vi "Create Measurement Client.vi"() -> ()   [LabVIEW 2021, in "MeasurementClient Editor.lvlib"]
uses:
  _MeasurementClient Utility/MeasurementClient Editor.lvlib
  <vilib>/Utility/error.llb/ErrWarn.ctl
  _MeasurementClient Utility/Refresh Button.ctl
  <vilib>/gRPC/Generated APIs/ni/measurementlink/discovery/v1/RPC Messages/ni_measurementlink_discovery_v1_EnumerateServicesRequest.ctl
  _MeasurementClient Utility/Data Holder.ctl
  <vilib>/gRPC/Generated APIs/ni/measurementlink/discovery/v1/RPC Messages/ni_measurementlink_discovery_v1_EnumerateServicesResponse.ctl
  <vilib>/gRPC/Generated APIs/ni/measurementlink/discovery/v1/RPC Messages/ni_measurementlink_discovery_v1_ServiceDescriptor.ctl
  <vilib>/gRPC/Generated APIs/ni/measurementlink/discovery/v1/RPC Messages/ni_measurementlink_discovery_v1_ServiceDescriptor_AnnotationsEntry.ctl
  <vilib>/Utility/miscctls.llb/LVRowAndColumnTypeDef.ctl
  _Generator Helpers/Generator Helpers.lvlib
  <vilib>/gRPC/Generated APIs/ni/measurementlink/discovery/v1/ni.measurementlink.discovery.v1.api.lvlib
  <vilib>/Plug-In SDKs/Clients/Discovery V1/NI Discovery V1 Client.lvlib
  Measurement V2 Client Generator Runtime/NI Measurement V2 Client Generator Runtime.lvlib
panel:
  in  "Tab Control":enum32{"Inputs", "Status"}(tab)
  in  "Select All":bool
  in  "Refresh":T1
  out "Active Project Name":string
  in  "Available Measurements":i32(listbox)=-1
  in  "Create Client":bool
  out "Warning":T2 caption="The selected measurement plug-in client name(s) already exists or contains invalid characters: \n \\ / : * ? \" < > |"
  out "Error Message":string
  in  "Client Status":i32(listbox)=-1 caption="Measurement Plug-In Client Creation Status"
  # "* Project in which the measurement plug-in client vi will be created"
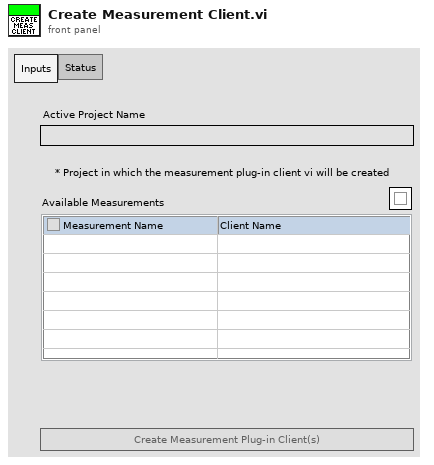
[diagram p1: front panel]
types:
  T1 = typedef "MeasurementClient Editor.lvlib/Refresh Button.ctl" = bool
  T2 = typedef "ErrWarn.ctl" = bool
  T3 = enum8{"Enabled", "Disabled", "Disabled and Grayed Out"}
  T4 = typedef "MeasurementClient Editor.lvlib/Data Holder.ctl" = cluster{"project ref":refnum<vi>, "multicolumnListbox ref":refnum<vi>, "available measurement details":T5, "statusListbox ref":refnum<vi>, "error messages":string[]}
  T5 = typedef "ni.measurementlink.discovery.v1.api.lvlib/ni_measurementlink_discovery_v1_EnumerateServicesResponse.ctl" = cluster{"available_services":T6[], "unreachable":string[]}
  T6 = typedef "ni.measurementlink.discovery.v1.api.lvlib/ni_measurementlink_discovery_v1_ServiceDescriptor.ctl" = cluster{"display_name":string, "description_url":string, "provided_interfaces":string[], "service_class":string, "annotations":T7[], "versions":string[]}
  T7 = typedef "ni.measurementlink.discovery.v1.api.lvlib/ni_measurementlink_discovery_v1_ServiceDescriptor_AnnotationsEntry.ctl" = cluster{"key":string, "value":string}
  T8 = typedef "ni.measurementlink.discovery.v1.api.lvlib/ni_measurementlink_discovery_v1_EnumerateServicesRequest.ctl" = cluster{"provided_interface":string, "service_class":string}
  T9 = typedef "LVRowAndColumnTypeDef.ctl" = cluster{"Row":i32, "Column":i32}
  T10 = typedef "MeasurementClient Editor.lvlib/Client Creation Status.ctl" = enum16{"Success", "Fail"}
  T11 = typedef "LVPoint32TypeDef.ctl" = cluster{"Horizontal":i32, "Vertical":i32}
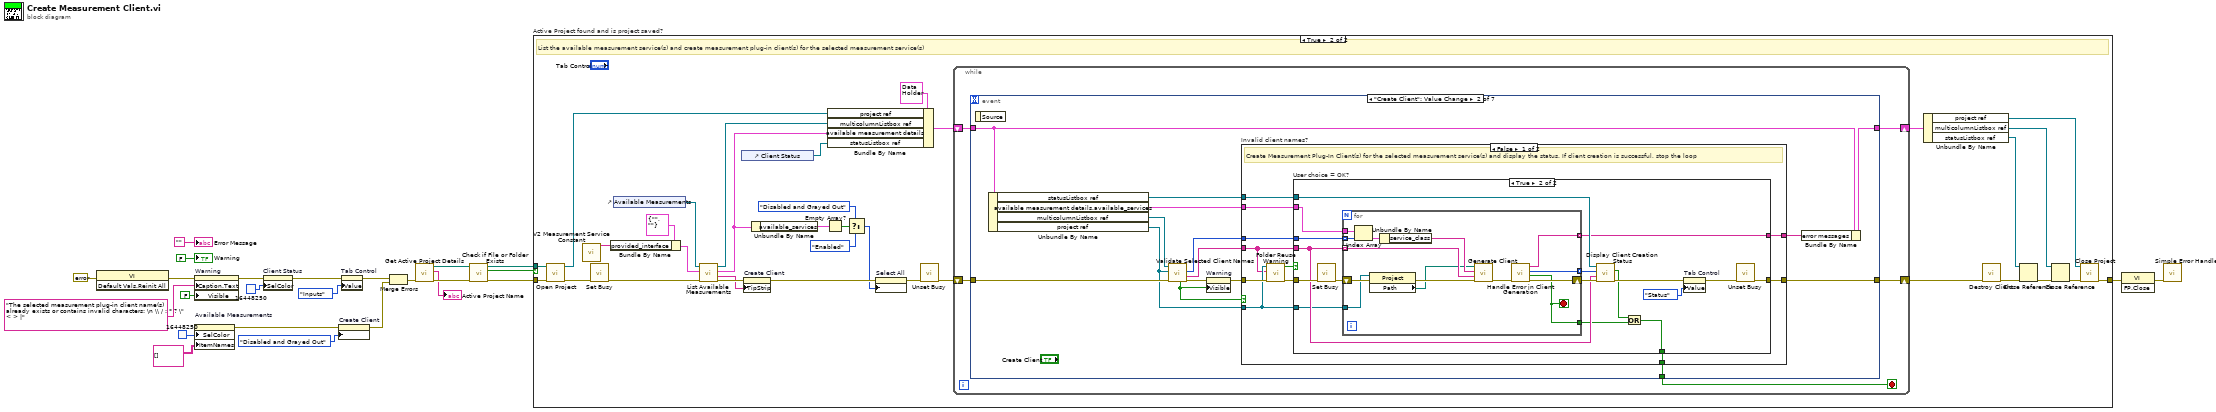
[diagram p0: block diagram]
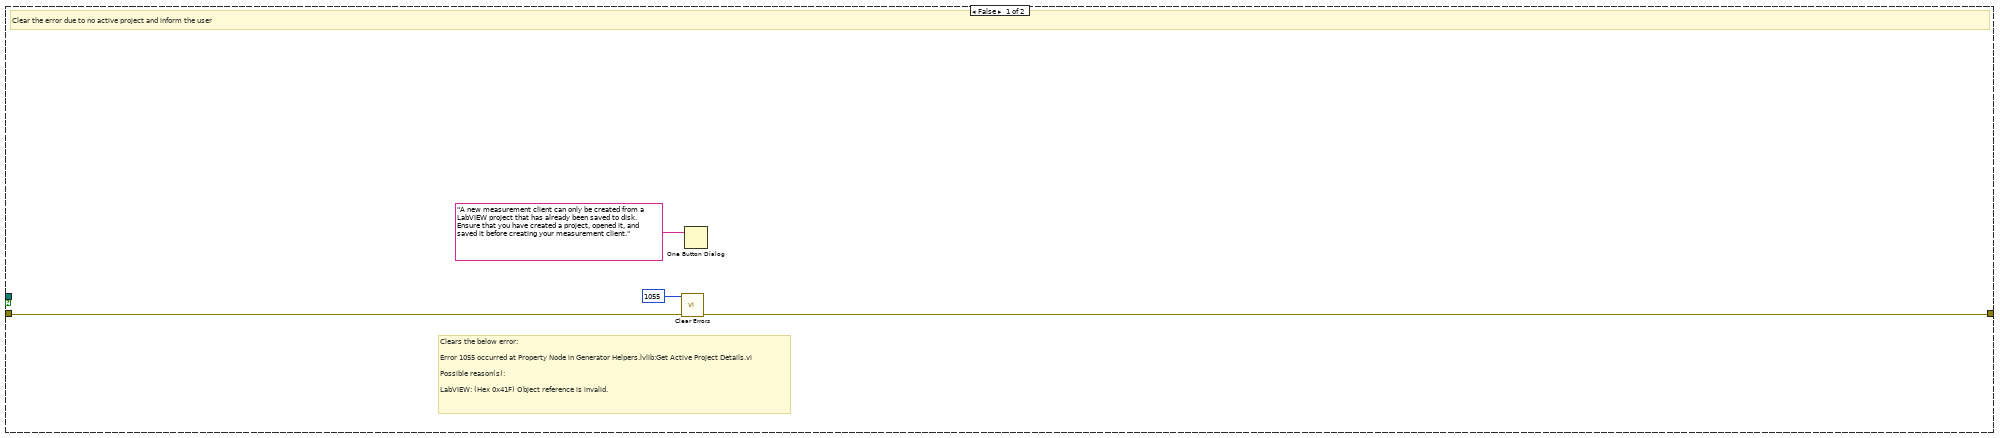
[diagram p2: hidden frame]
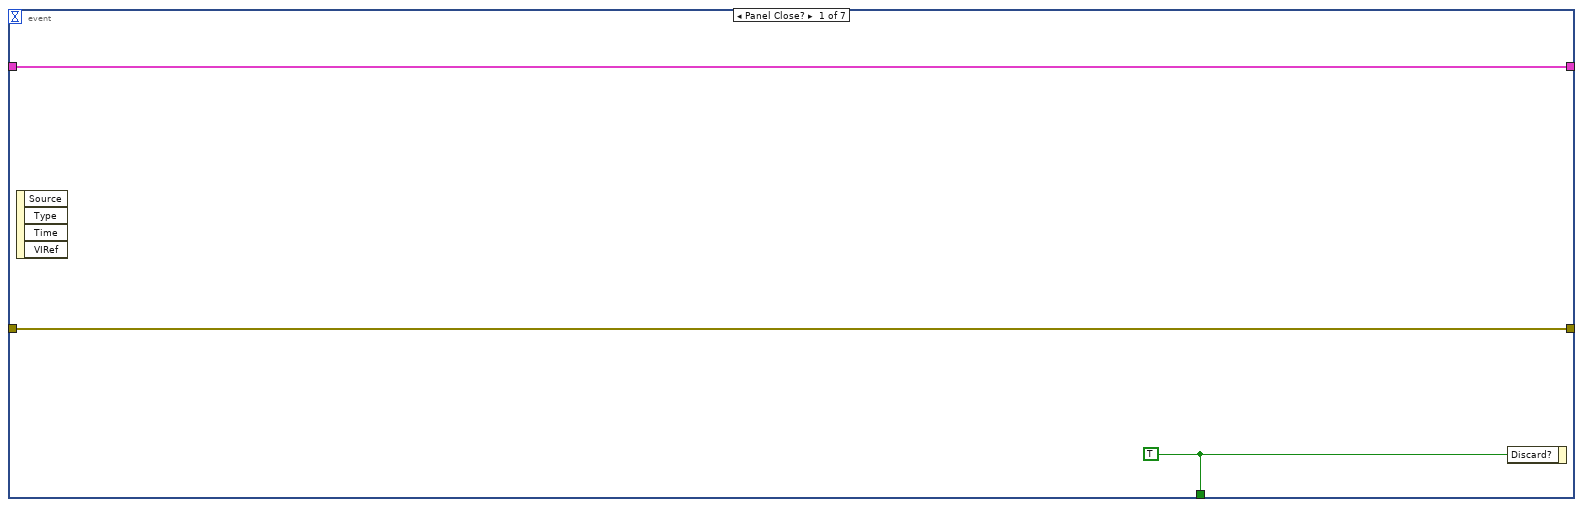
[diagram p3: hidden frame]
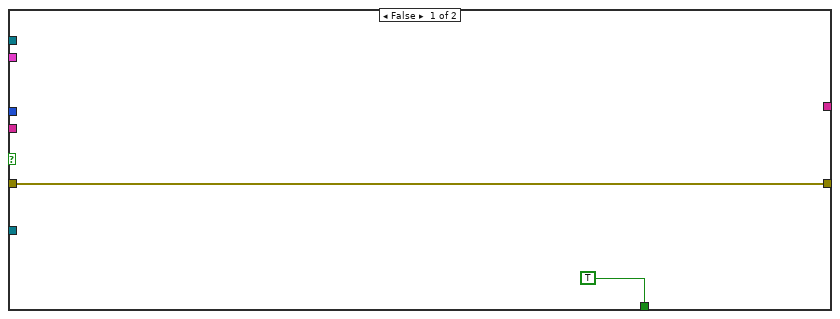
[diagram p4: hidden frame]
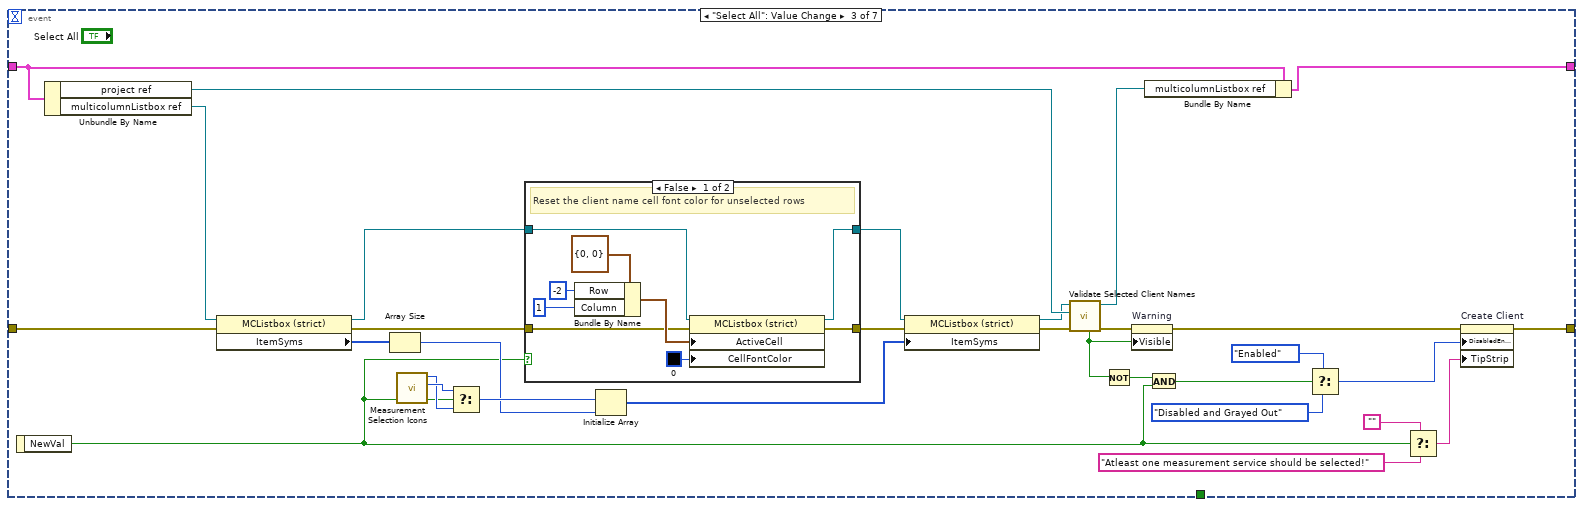
[diagram p6: hidden frame]
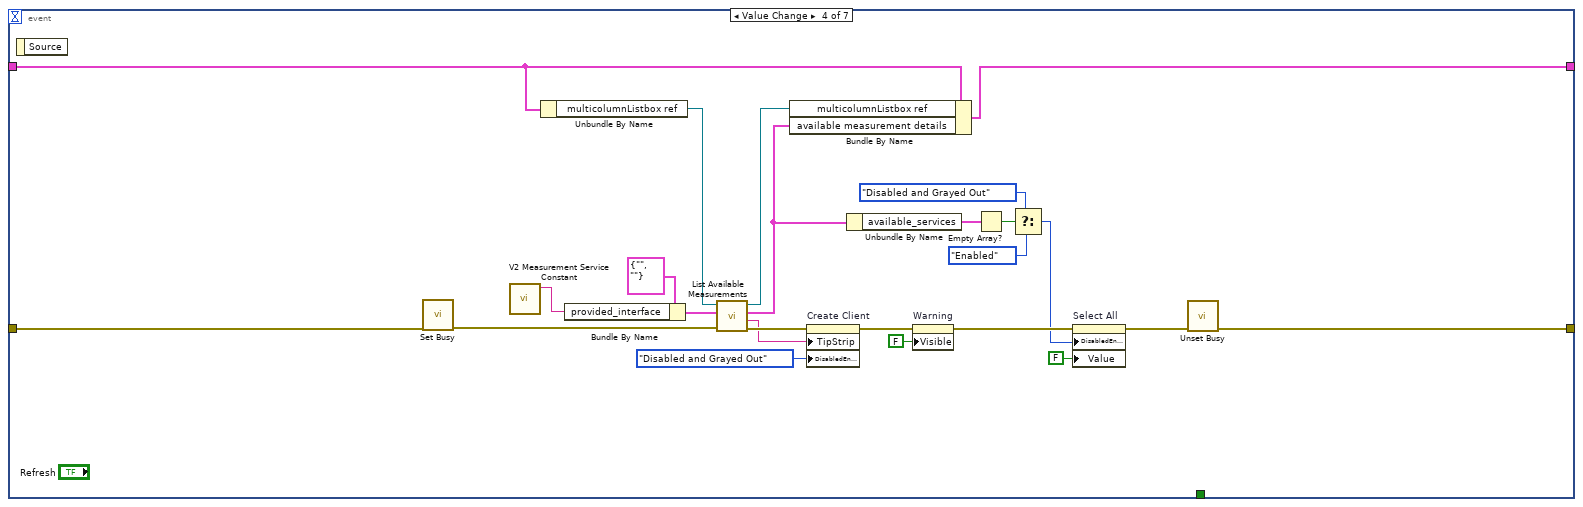
[diagram p8: hidden frame]
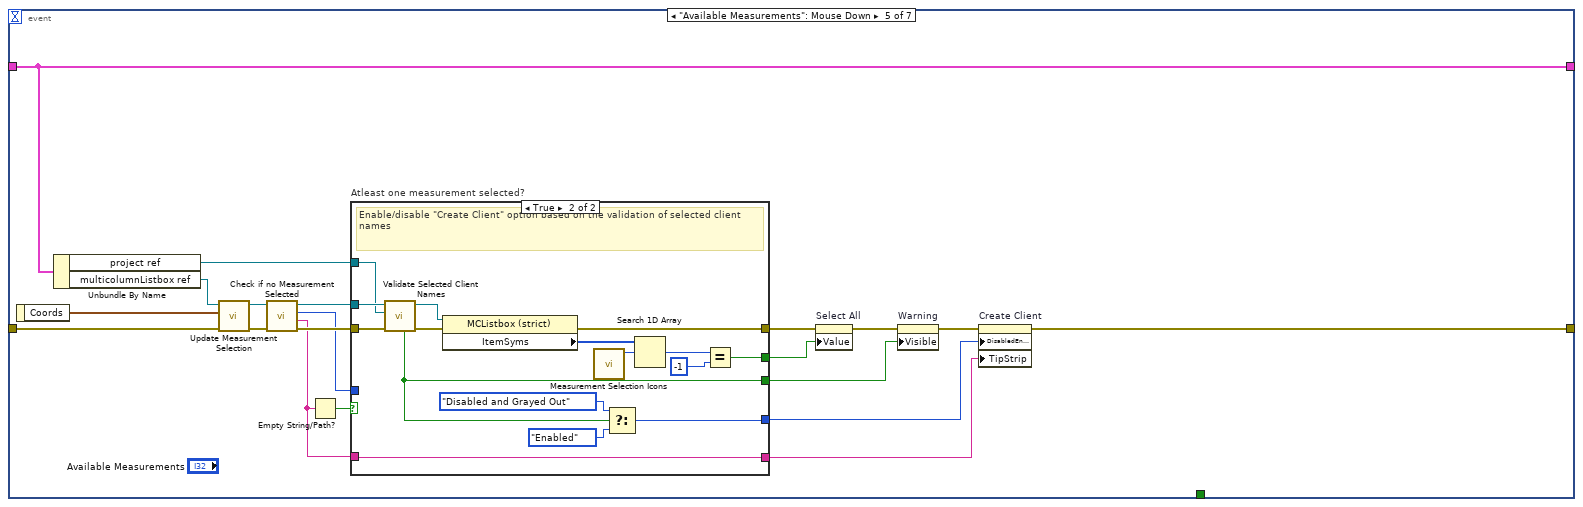
[diagram p9: hidden frame]
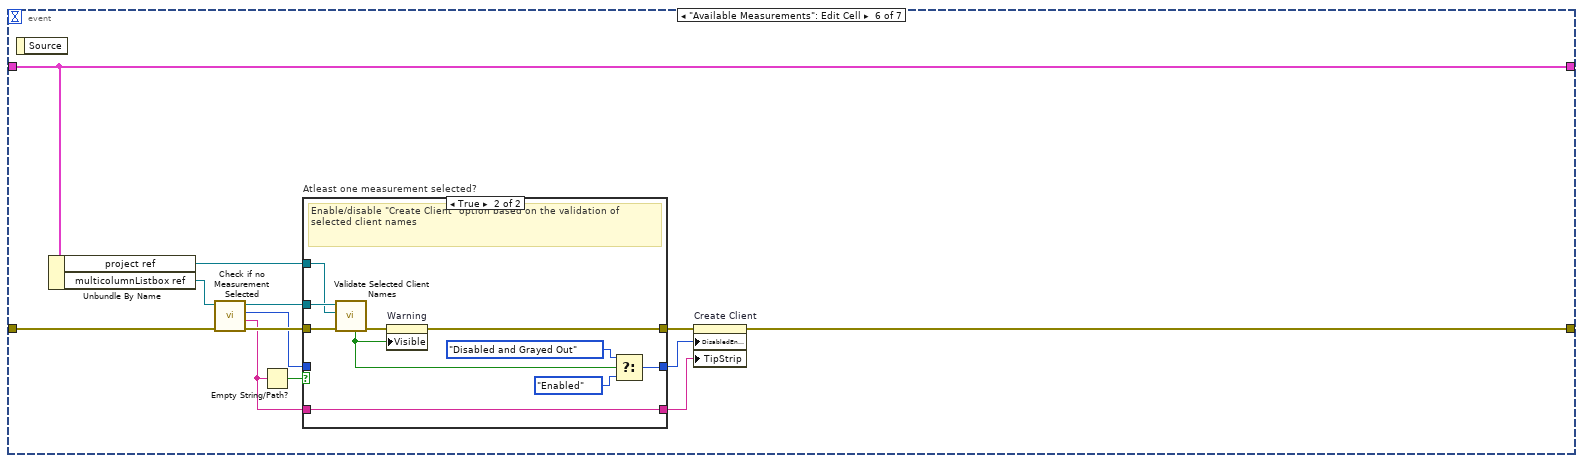
[diagram p11: hidden frame]
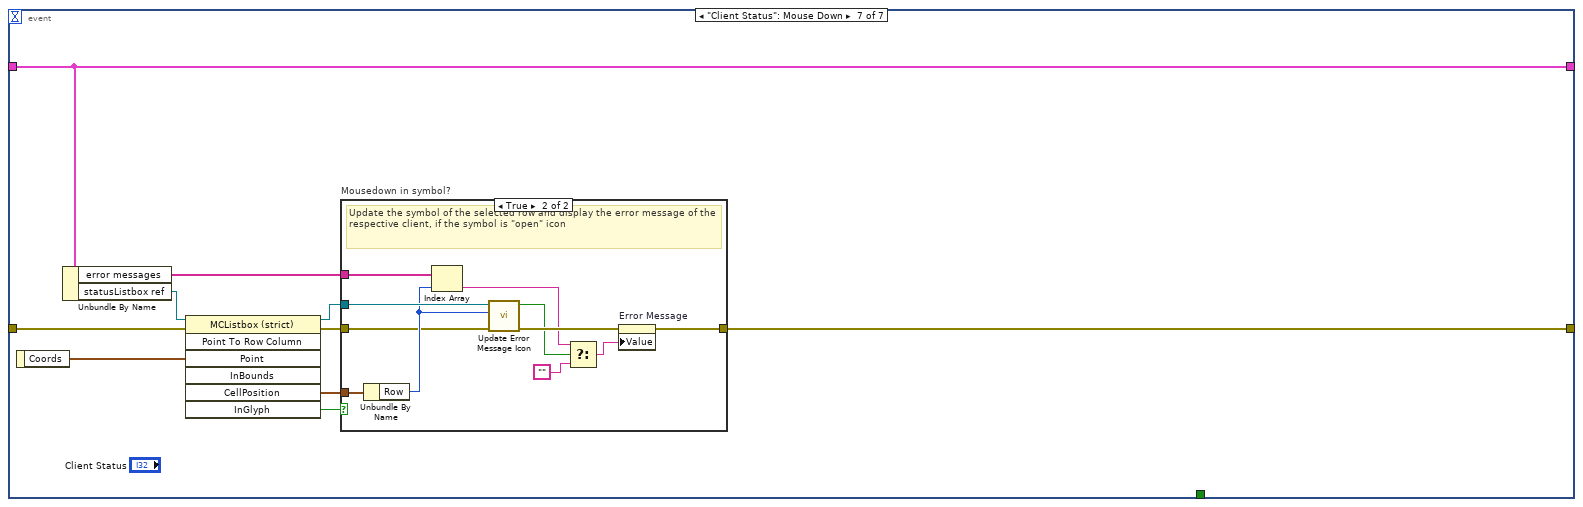
[diagram p13: hidden frame]
diagram:
  n1 = invoke class="VI" method="Default Vals.Reinit All"(error in=errorcluster {"status"=FALSE, "code"=0, "source"=""} ("error in (no error)")) -> (error out=w19:errorcluster)  [unwired: 2 in, 2 out]
  n2 = property on="Warning" class="Bool"(error in=w19, "Caption.Text"="The selected measurement plug-in client name(s) already exists or contains invalid characters: \n \\ / : * ? \" < > |" ("Status"), "Visible"=FALSE) -> (error out=w12:errorcluster)  [unwired: 1 in, 1 out]
  n3 = property on="Available Measurements" class="MCListbox (strict)"("SelColor"=u32 16448250 ("Selection Color"), "ItemNames"=string[][] [] ("Item Names")) -> (error out=w9:errorcluster)  [unwired: 2 in, 1 out]
  n4 = property on="Client Status" class="MCListbox (strict)"(error in=w12, "SelColor"=u32 16448250 ("Selection Color")) -> (error out=w13:errorcluster)  [unwired: 1 in, 1 out]
  n5 = property on="Create Client" class="Bool"(error in=w9, "DisabledEnum"=T3."Disabled and Grayed Out" ("Disabled")) -> (error out=w8:errorcluster)  [unwired: 1 in, 1 out]
  n6 = property on="Tab Control" class="TabCtl (strict)"(error in=w13, "Value"=enum32{"Inputs", "Status"}."Inputs" ("Tab Control")) -> (error out=w11:errorcluster)  [unwired: 1 in, 1 out]
  n7 = Merge Errors(w11, w8) -> (w7:errorcluster)
  n8 = call "Get Active Project Details.vi"("error in"=w7) -> ("error out"=w6:errorcluster, "name"=→"Active Project Name":string, "path"=w5:path)  [unwired: 8 in]
  n9 = call <vilib>:"Check if File or Folder Exists.vi"("error in (no error)"=w6, "path"=w5) -> ("error out"=w2:errorcluster, "file or folder exists?"=w1:bool, "dup path"=w3:path)  [unwired: 7 in]
  n10 = case "Active Project found and is project saved?" shown="True" w1 {
    tunnel: [w29 w47] -> w23
    tunnel: w3 -> [_ w62]
    tunnel: w2 -> [w26 w56]
    frame False {
      # "Clears the below error:\n\nError 1055 occurred at Property Node in Generator Helpers.lvlib:Get Active Project Details.vi\n\nPossible reason(s):\n\nLabVIEW: (Hex 0x41F) Object reference is invalid."
      # "Clear the error due to no active project and inform the user"
      n11 = call <vilib>:"Clear Errors.vi"("error in (no error)"=w26, "specific error code to clear (0: all)"=1055) -> ("error out"=w29:errorcluster)  [unwired: 4 in, 1 out]
      n12 = One Button Dialog(message="A new measurement client can only be created from a LabVIEW project that has already been saved to disk.  Ensure that you have created a project, opened it, and saved it before creating your measurement client.") -> ()  [unwired: 1 in, 1 out]
    }
    frame True {
      # "List the available measurement service(s) and create measurement plug-in client(s) for the selected measurement service(s)"
      n13 = call "Open Project.vi"("error in"=w56, "path"=w62) -> ("error out"=w57:errorcluster, "project ref"=w51:refnum<vi>)  [unwired: 8 in]
      n14 = call "V2 Measurement Service Constant.vi"() -> ("provided_interface"=w39:string)  [unwired: 11 in]
      n15 = call <vilib>:"Set Busy.vi"("error in (no error)"=w57) -> ("error out"=w59:errorcluster)  [unwired: 9 in, 1 out]
      n16 = Bundle By Name(cluster=T8 {"provided_interface"="", "service_class"=""} ("request data"), "provided_interface"=w39) -> (w40:T8)
      n17 = control-ref of="Available Measurements"() -> (w49:refnum<vi>)
      n18 = call "List Available Measurements.vi"("error in (no error)"=w59, "enumerate services request"=w40, "multicolumnListbox ref in"=w49) -> ("error out"=w60:errorcluster, "warning"=w53:string, "available measurement details"=w36:T5, "multicolumnListbox ref"=w50:refnum<vi>)  [unwired: 5 in]
      n19 = control-ref of="Client Status"() -> (w30:refnum<vi>)
      n20 = property on="Create Client" class="Bool"(error in=w60, "TipStrip"=w53) -> (error out=w38:errorcluster)  [unwired: 1 in, 1 out]
      n21 = Unbundle By Name(w36) -> ("available_services"=w35:T6[])
      n22 = Empty Array?(array=w35) -> (empty?=w32:bool)
      n23 = Bundle By Name(cluster=T4 {"project ref"=refnum, "multicolumnListbox ref"=refnum, "available measurement details"={"available_services"=[], "unreachable"=[]}, "statusListbox ref"=refnum, "error messages"=[]}, "project ref"=w51, "multicolumnListbox ref"=w50, "available measurement details"=w36, "statusListbox ref"=w30) -> (w48:T4)
      n24 = Select(t=T3."Disabled and Grayed Out" ("Disabled"), s=w32, f=T3."Enabled" ("Disabled")) -> (s? t:f=w31:T3)
      n25 = property on="Select All" class="Bool (strict)"(error in=w38, "DisabledEnum"=w31) -> (error out=w37:errorcluster)  [unwired: 1 in, 1 out]
      n26 = call <vilib>:"Unset Busy.vi"("error in (no error)"=w37) -> ("error out"=w58:errorcluster)  [unwired: 10 in]
      n27 = while {
        shift-right: [w66] -> w43
        shift-left: w58 -> [w67]
        shift-right: [w64] -> w54
        shift-left: w48 -> [w65]
        stop <- w63 stop-if-true
        n28 = event shown="[1] \"Create Client\": Value Change" {
          selector: _ -> [_ _ _ _ _ _ _]
          dyn-events: _ -> [_ _ _ _ _ _ _]
          timeout: _ -> [_ _ _ _ _ _ _]
          tunnel: w67 -> [w70 w85 w140 w185 w211 w237 w268]
          tunnel: [w70 w75 w149 w182 w210 w247 w271] -> w66
          tunnel: w65 -> [w69 w80 w147 w193 w216 w248 w269]
          tunnel: [w69 w77 w145 w191 w216 w248 w269] -> w64
          tunnel: [w68 w72 _ _ _ _ _] -> w63
          event Panel Close? {
            w68 = TRUE ("Discard?")
            # "Discard panel close and stop the execution of measurement plug-in client generator"
            n29 = event-data() -> ()  [unwired: 1 in, 4 out]
            n30 = event-data("Discard?"=w68) -> ()  [unwired: 1 in, 1 out]
          }
          event "Create Client": Value Change {
            # "Validate client name and create measurement plug-in client for the selected measurement service(s), if no invalid client name"
            n31 = event-data() -> ()  [unwired: 1 in, 1 out]
            n32 = Unbundle By Name(w80) -> ("statusListbox ref"=w78:refnum<vi>, "available measurement details.available_services"=w76:T6[], "multicolumnListbox ref"=w84:refnum<vi>, "project ref"=w79:refnum<vi>)
            n33 = call "Validate Selected Client Names.vi"("error in (no error)"=w85, "project ref"=w79, "multicolumnListbox in"=w84) -> ("error out"=w83:errorcluster, "selected client names"=w74:string[], "selected measurement indices"=w81:i32[], "warning?"=w73:bool)  [unwired: 4 in, 1 out]
            n34 = property on="Warning" class="Bool"(error in=w83, "Visible"=w73) -> (error out=w82:errorcluster)  [unwired: 1 in, 1 out]
            n35 = case "Invalid client names?" shown="False" w73 {
              tunnel: w82 -> [w96 w130]
              tunnel: w81 -> [w95 _]
              tunnel: w79 -> [w89 _]
              tunnel: [w92 w130] -> w75
              tunnel: w78 -> [w94 _]
              tunnel: w76 -> [w93 _]
              tunnel: w74 -> [w87 _]
              tunnel: [w91 _] -> w72
              tunnel: [w86 _] -> w71
              frame False {
                # "Create Measurement Plug-In Client(s) for the selected measurement service(s) and display the status. If client creation is successful, stop the loop"
                n36 = call "Folder Reuse Warning.vi"("error in"=w96, "folder names"=w87, "project ref"=w89) -> ("error out"=w90:errorcluster, "proceed?"=w88:bool)  [unwired: 7 in]
                n37 = case "User choice = OK?" shown="True" w88 {
                  tunnel: w95 -> [_ w115]
                  tunnel: w94 -> [_ w112]
                  tunnel: w93 -> [_ w111]
                  tunnel: [w98 w107] -> w92
                  tunnel: [TRUE ("all success?") w102] -> w91
                  tunnel: w90 -> [w98 w106]
                  tunnel: w87 -> [_ w105]
                  tunnel: w89 -> [_ w104]
                  tunnel: [_ w99] -> w86
                  frame False {
                  }
                  frame True {
                    n38 = call <vilib>:"Set Busy.vi"("error in (no error)"=w106) -> ("error out"=w114:errorcluster)  [unwired: 9 in, 1 out]
                    n39 = for {
                      tunnel: w111 -> [w129]
                      shift-right: [w119] -> w113
                      shift-left: w114 -> [w126]
                      tunnel: w115 -> [w127] mode=indexing
                      tunnel: w104 -> [w122]
                      tunnel: w105 -> [w124] mode=indexing
                      tunnel: [w118] -> w99 mode=indexing
                      tunnel: [w117] -> w101 mode=indexing
                      tunnel: [w116] -> w100
                      stop <- w116 stop-if-true
                      n40 = Index Array(array=w129, index=w127) -> (element=w128:T6)
                      n41 = property class="Project"(reference=w122, error in=w126) -> (error out=w123:errorcluster, "Path"=w121:path)  [unwired: 1 out]
                      n42 = Unbundle By Name(w128) -> ("service_class"=w125:string)
                      n43 = call "Generate Client.vi"("error in"=w123, "client name"=w124, "service class"=w125, "project path"=w121) -> ("error out"=w120:errorcluster)  [unwired: 7 in]
                      n44 = call "Handle Error in Client Generation.vi"("error in"=w120) -> ("error out"=w119:errorcluster, "InstrumentStudio Pro < Q4?"=w116:bool, "status"=w117:T10, "error message"=w118:string)  [unwired: 7 in]
                    }
                    n45 = call "Display Client Creation Status.vi"("error in"=w113, "client names"=w105, "status"=w101, "statusListbox in"=w112) -> ("error out"=w109:errorcluster, "all success?"=w103:bool)  [unwired: 5 in, 1 out]
                    n46 = Or(x=w103, y=w100) -> (x .or. y?=w102:bool)
                    n47 = property on="Tab Control" class="TabCtl (strict)"(error in=w109, "Value"=enum32{"Inputs", "Status"}."Status" ("Tab Control")) -> (error out=w108:errorcluster)  [unwired: 1 in, 1 out]
                    n48 = call <vilib>:"Unset Busy.vi"("error in (no error)"=w108) -> ("error out"=w107:errorcluster)  [unwired: 10 in]
                  }
                }
              }
              frame True {
                # "Pass"
              }
            }
            n49 = Bundle By Name(cluster=w80, "error messages"=w71) -> (w77:T4)
          }
          event "Select All": Value Change {
            n50 = event-data() -> ("NewVal"=w132:bool)  [unwired: 1 in]
            n51 = Unbundle By Name(w147) -> ("project ref"=w148:refnum<vi>, "multicolumnListbox ref"=w161:refnum<vi>)
            n52 = property class="MCListbox (strict)"(reference=w161, error in=w140) -> (reference out=w144:refnum<vi>, error out=w139:errorcluster, "ItemSyms"=w135:i32[])
            n53 = Array Size(array=w135) -> (size(s)=w133:i32)
            n54 = call "Measurement Selection Icons.vi"() -> ("Checked"=w137:i32, "Unchecked"=w136:i32)  [unwired: 10 in]
            n55 = Select(t=w137, s=w132, f=w136) -> (s? t:f=w134:i32)
            n56 = case shown="False" w132 {
              tunnel: w144 -> [w166 w172]
              tunnel: [w165 w172] -> w142
              tunnel: w139 -> [w164 w171]
              tunnel: [w163 w171] -> w138
              frame False {
                # "Reset the client name cell font color for unselected rows"
                n57 = Bundle By Name(cluster=T9 {"Row"=0, "Column"=0} ("Active Cell:Active Cell"), "Row"=-2, "Column"=1) -> (w168:T9)
                n58 = property class="MCListbox (strict)"(reference=w166, error in=w164, "ActiveCell"=w168, "CellFontColor"=u32 0 ("Active Cell:Cell Font:Color")) -> (reference out=w165:refnum<vi>, error out=w163:errorcluster)
              }
              frame True {
                # "Pass"
              }
            }
            n59 = Initialize Array(w134, w133) -> (w131:i32[])
            n60 = property class="MCListbox (strict)"(reference=w142, error in=w138, "ItemSyms"=w131) -> (reference out=w141:refnum<vi>, error out=w143:errorcluster)
            n61 = call "Validate Selected Client Names.vi"("error in (no error)"=w143, "project ref"=w148, "multicolumnListbox in"=w141) -> ("error out"=w160:errorcluster, "multicolumnListbox out"=w146:refnum<vi>, "warning?"=w158:bool)  [unwired: 4 in, 2 out]
            n62 = Not(x=w158) -> (.not. x?=w157:bool)
            n63 = property on="Warning" class="Bool"(error in=w160, "Visible"=w158) -> (error out=w159:errorcluster)  [unwired: 1 in, 1 out]
            n64 = Bundle By Name(cluster=w147, "multicolumnListbox ref"=w146) -> (w145:T4)
            n65 = And(x=w157, y=w132) -> (x .and. y?=w156:bool)
            n66 = Select(t=T3."Enabled" ("Disabled"), s=w156, f=T3."Disabled and Grayed Out" ("Disabled")) -> (s? t:f=w153:T3)
            n67 = Select(t="", s=w132, f="Atleast one measurement service should be selected!") -> (s? t:f=w150:string)
            n68 = property on="Create Client" class="Bool"(error in=w159, "DisabledEnum"=w153, "TipStrip"=w150) -> (error out=w149:errorcluster)  [unwired: 1 in, 1 out]
          }
          event Value Change {
            n69 = event-data() -> ()  [unwired: 1 in, 1 out]
            n70 = call <vilib>:"Set Busy.vi"("error in (no error)"=w185) -> ("error out"=w184:errorcluster)  [unwired: 9 in, 1 out]
            n71 = call "V2 Measurement Service Constant.vi"() -> ("provided_interface"=w195:string)  [unwired: 11 in]
            n72 = Unbundle By Name(w193) -> ("multicolumnListbox ref"=w189:refnum<vi>)
            n73 = Bundle By Name(cluster=T8 {"provided_interface"="", "service_class"=""} ("request data"), "provided_interface"=w195) -> (w183:T8)
            n74 = call "List Available Measurements.vi"("error in (no error)"=w184, "enumerate services request"=w183, "multicolumnListbox ref in"=w189) -> ("error out"=w194:errorcluster, "warning"=w190:string, "available measurement details"=w177:T5, "multicolumnListbox ref"=w192:refnum<vi>)  [unwired: 5 in]
            n75 = Bundle By Name(cluster=w193, "multicolumnListbox ref"=w192, "available measurement details"=w177) -> (w191:T4)
            n76 = property on="Create Client" class="Bool"(error in=w194, "TipStrip"=w190, "DisabledEnum"=T3."Disabled and Grayed Out" ("Disabled")) -> (error out=w187:errorcluster)  [unwired: 1 in, 1 out]
            n77 = Unbundle By Name(w177) -> ("available_services"=w181:T6[])
            n78 = property on="Warning" class="Bool"(error in=w187, "Visible"=FALSE) -> (error out=w176:errorcluster)  [unwired: 1 in, 1 out]
            n79 = Empty Array?(array=w181) -> (empty?=w178:bool)
            n80 = Select(t=T3."Disabled and Grayed Out" ("Disabled"), s=w178, f=T3."Enabled" ("Disabled")) -> (s? t:f=w174:T3)
            n81 = property on="Select All" class="Bool (strict)"(error in=w176, "DisabledEnum"=w174, "Value"=FALSE ("Select All")) -> (error out=w175:errorcluster)  [unwired: 1 in, 1 out]
            n82 = call <vilib>:"Unset Busy.vi"("error in (no error)"=w175) -> ("error out"=w182:errorcluster)  [unwired: 10 in]
          }
          event "Available Measurements": Mouse Down {
            # "Update the selection of measurement service and enable/disable \"Create Client\" accordingly"
            n83 = event-data() -> ("Coords"=w209:T11)  [unwired: 1 in]
            n84 = Unbundle By Name(w216) -> ("project ref"=w202:refnum<vi>, "multicolumnListbox ref"=w215:refnum<vi>)
            n85 = call "Update Measurement Selection.vi"("error in (no error)"=w211, "mouseDown coords"=w209, "multicolumnListbox in"=w215) -> ("error out"=w213:errorcluster, "multicolumnListbox out"=w214:refnum<vi>)  [unwired: 7 in]
            n86 = call "Check if no Measurement Selected.vi"("error in (no error)"=w213, "multicolumnListbox in"=w214) -> ("error out"=w212:errorcluster, "warning?"=w203:string, "create client disabled?"=w205:T3, "multicolumnListbox out"=w208:refnum<vi>)  [unwired: 6 in]
            n87 = Empty String/Path?(string/path=w203) -> (empty?=w207:bool)
            n88 = case "Atleast one measurement selected?" shown="True" w207 {
              tunnel: w212 -> [w219 w230]
              tunnel: [w219 w227] -> w199
              tunnel: w208 -> [_ w232]
              tunnel: [w218 w233] -> w204
              tunnel: w203 -> [w218 w233]
              tunnel: [w217 w234] -> w206
              tunnel: w205 -> [w217 _]
              tunnel: w202 -> [_ w231]
              tunnel: [_ w229] -> w200
              tunnel: [_ w221] -> w197
              frame False {
                # "Enable/disable the \"Create Client\" option based on measurement selection"
              }
              frame True {
                # "Enable/disable \"Create Client\" option based on the validation of selected client names"
                n89 = call "Validate Selected Client Names.vi"("error in (no error)"=w230, "project ref"=w231, "multicolumnListbox in"=w232) -> ("error out"=w228:errorcluster, "multicolumnListbox out"=w226:refnum<vi>, "warning?"=w229:bool)  [unwired: 4 in, 2 out]
                n90 = property class="MCListbox (strict)"(reference=w226, error in=w228) -> (error out=w227:errorcluster, "ItemSyms"=w224:i32[])  [unwired: 1 out]
                n91 = call "Measurement Selection Icons.vi"() -> ("Unchecked"=w220:i32)  [unwired: 10 in, 1 out]
                n92 = Select(t=T3."Disabled and Grayed Out" ("Disabled"), s=w229, f=T3."Enabled") -> (s? t:f=w234:T3)
                n93 = Search 1D Array(1D array=w224, element=w220) -> (index of element=w223:i32)  [unwired: 1 in]
                n94 = Equal?(x=w223, y=-1) -> (x = y?=w221:bool)
              }
            }
            n95 = property on="Select All" class="Bool (strict)"(error in=w199, "Value"=w197) -> (error out=w198:errorcluster)  [unwired: 1 in, 1 out]
            n96 = property on="Warning" class="Bool"(error in=w198, "Visible"=w200) -> (error out=w201:errorcluster)  [unwired: 1 in, 1 out]
            n97 = property on="Create Client" class="Bool"(error in=w201, "DisabledEnum"=w206, "TipStrip"=w204) -> (error out=w210:errorcluster)  [unwired: 1 in, 1 out]
          }
          event "Available Measurements": Edit Cell {
            n98 = event-data() -> ()  [unwired: 1 in, 1 out]
            n99 = Unbundle By Name(w248) -> ("project ref"=w238:refnum<vi>, "multicolumnListbox ref"=w236:refnum<vi>)
            n100 = call "Check if no Measurement Selected.vi"("error in (no error)"=w237, "multicolumnListbox in"=w236) -> ("error out"=w243:errorcluster, "warning?"=w239:string, "create client disabled?"=w241:T3, "multicolumnListbox out"=w244:refnum<vi>)  [unwired: 6 in]
            n101 = Empty String/Path?(string/path=w239) -> (empty?=w242:bool)
            n102 = case "Atleast one measurement selected?" shown="True" w242 {
              tunnel: [w250 w253] -> w246
              tunnel: [w251 w259] -> w245
              tunnel: w244 -> [_ w258]
              tunnel: w243 -> [w250 w254]
              tunnel: w241 -> [w251 _]
              tunnel: [w249 w257] -> w240
              tunnel: w239 -> [w249 w257]
              tunnel: w238 -> [_ w256]
              frame False {
                # "Enable/disable the \"Create Client\" option based on measurement selection"
              }
              frame True {
                # "Enable/disable \"Create Client\" option based on the validation of selected client names"
                n103 = call "Validate Selected Client Names.vi"("error in (no error)"=w254, "project ref"=w256, "multicolumnListbox in"=w258) -> ("error out"=w255:errorcluster, "warning?"=w252:bool)  [unwired: 4 in, 3 out]
                n104 = property on="Warning" class="Bool"(error in=w255, "Visible"=w252) -> (error out=w253:errorcluster)  [unwired: 1 in, 1 out]
                n105 = Select(t=T3."Disabled and Grayed Out" ("Disabled"), s=w252, f=T3."Enabled") -> (s? t:f=w259:T3)
              }
            }
            n106 = property on="Create Client" class="Bool"(error in=w246, "DisabledEnum"=w245, "TipStrip"=w240) -> (error out=w247:errorcluster)  [unwired: 1 in, 1 out]
          }
          event "Client Status": Mouse Down {
            n107 = event-data() -> ("Coords"=w265:T11)  [unwired: 1 in]
            n108 = Unbundle By Name(w269) -> ("error messages"=w270:string[], "statusListbox ref"=w266:refnum<vi>)
            n109 = invoke class="MCListbox (strict)" method="Point To Row Column"(reference=w266, error in=w268, "Point"=w265) -> (reference out=w263:refnum<vi>, error out=w267:errorcluster, "CellPosition"=w264:T9, "InGlyph"=w262:bool)  [unwired: 4 in, 3 out]
            n110 = case "Mousedown in symbol?" shown="True" w262 {
              tunnel: [w272 w277] -> w271
              tunnel: w264 -> [_ w283]
              tunnel: w270 -> [_ w282]
              tunnel: w267 -> [w272 w279]
              tunnel: w263 -> [_ w281]
              frame False {
                # "Pass"
              }
              frame True {
                # "Update the symbol of the selected row and display the error message of the respective client, if the symbol is \"open\" icon"
                n111 = Unbundle By Name(w283) -> ("Row"=w280:i32)
                n112 = Index Array(array=w282, index=w280) -> (element=w275:string)
                n113 = call "Update Error Message Icon.vi"("error in"=w279, "selected row"=w280, "statusListbox in"=w281) -> ("error out"=w278:errorcluster, "open?"=w276:bool)  [unwired: 7 in]
                n114 = Select(t=w275, s=w276, f="") -> (s? t:f=w273:string)
                n115 = property on="Error Message" class="Str"(error in=w278, "Value"=w273) -> (error out=w277:errorcluster)  [unwired: 1 in, 1 out]
              }
            }
          }
        }
      }
      n116 = Unbundle By Name(w54) -> ("project ref"=w55:refnum<vi>, "multicolumnListbox ref"=w61:refnum<vi>, "statusListbox ref"=w44:refnum<vi>)
      n117 = call <vilib>:"Destroy Client.vi"("error in"=w43) -> ("error out"=w42:errorcluster)  [unwired: 10 in]
      n118 = Close Reference(reference=w44, error in (no error)=w42) -> (error out=w45:errorcluster)
      n119 = Close Reference(reference=w61, error in (no error)=w45) -> (error out=w46:errorcluster)
      n120 = call "Close Project.vi"("error in"=w46, "project ref"=w55) -> ("error out"=w47:errorcluster)  [unwired: 9 in]
    }
  }
  n121 = invoke class="VI" method="FP.Close"(error in=w23) -> (error out=w25:errorcluster)  [unwired: 2 in, 2 out]
  n122 = call <vilib>:"Simple Error Handler.vi"("error in (no error)"=w25) -> ()  [unwired: 4 in, 5 out]
  "Warning" <- T2 FALSE ("Warning")
  "Error Message" <- ""
